vi "onTestDiscovery.vi"(8 "error in (no error)":errorcluster, 11 "Test Runner.Collection in":refnum<class "Test Runner.Collection.lvclass">) -> (0 "error out":errorcluster, 2 "Tests VIs":path[](array[path]), 3 "Test Runner.Collection out":refnum<class "Test Runner.Collection.lvclass">)   [LabVIEW 2020, in "Caraya.lvlib" / "Test Runner.Collection.lvclass"]
uses:
  Test Runner.Collection.lvclass
  Test Runner.Collection.lvclass/Test Runner.Collection.ctl
  Test Runner/Test Runner.lvclass
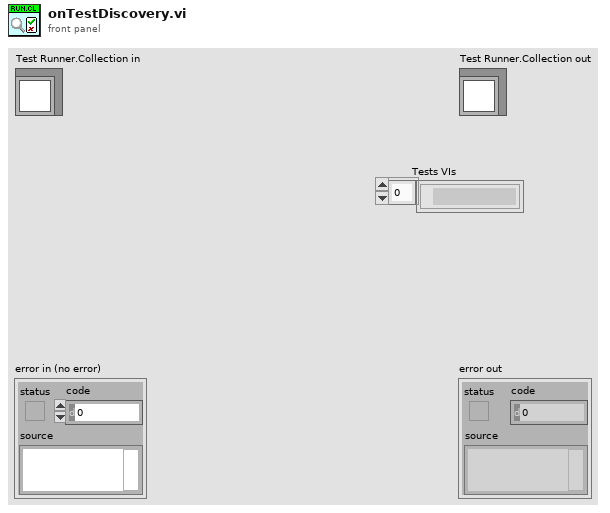
[diagram p1: front panel]
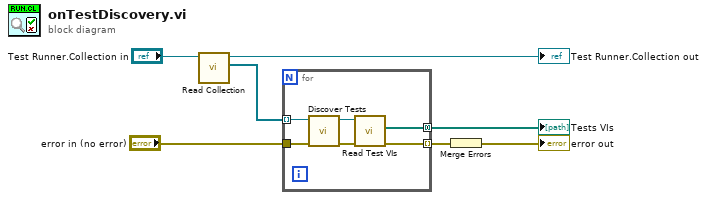
[diagram p0: block diagram]
diagram:
  n1 = call "Read Collection.vi"("Test Runner.Collection in"="Test Runner.Collection in") -> ("Test Runners"=w3:refnum<class "Test Runner.lvclass">[], "Test Runner.Collection out"=→"Test Runner.Collection out":refnum<class "Test Runner.Collection.lvclass">)  [unwired: 9 in]
  n2 = for {
    tunnel: [w9] -> w6 mode=concatenating
    tunnel: w3 -> [w8] mode=indexing
    tunnel: "error in (no error)" -> [w13]
    tunnel: [w10] -> w7 mode=indexing
    n3 = call "Discover Tests.vi"("error in (no error)"=w13, "Test Runner in"=w8) -> ("error out"=w11:errorcluster, "Test Runner out"=w12:refnum<class "Test Runner.lvclass">)  [unwired: 8 in]
    n4 = call "Read Test VIs.vi"("error in (no error)"=w11, "Test Runner in"=w12) -> ("error out"=w10:errorcluster, "Test VIs"=w9:path[])  [unwired: 7 in, 1 out]
  }
  "Tests VIs" <- w6
  n5 = Merge Errors(w7) -> (→"error out":errorcluster)
